vi "SaveMeasurement.vi"(8 "references":T1, 11 "measurement":T2) -> (0 "references out":T1, 3 "data":string[](array[string]))   [LabVIEW 2011]
doc: "Save measured data into the temporary .csv file for the case of program error."
uses:
  Measurement References.ctl
  <vilib>/Utility/NIReport.llb/NI_report.lvclass
  <vilib>/Utility/file.llb/Write To Spreadsheet File (string).vi
  <vilib>/Analysis/NI_AALBase.lvlib
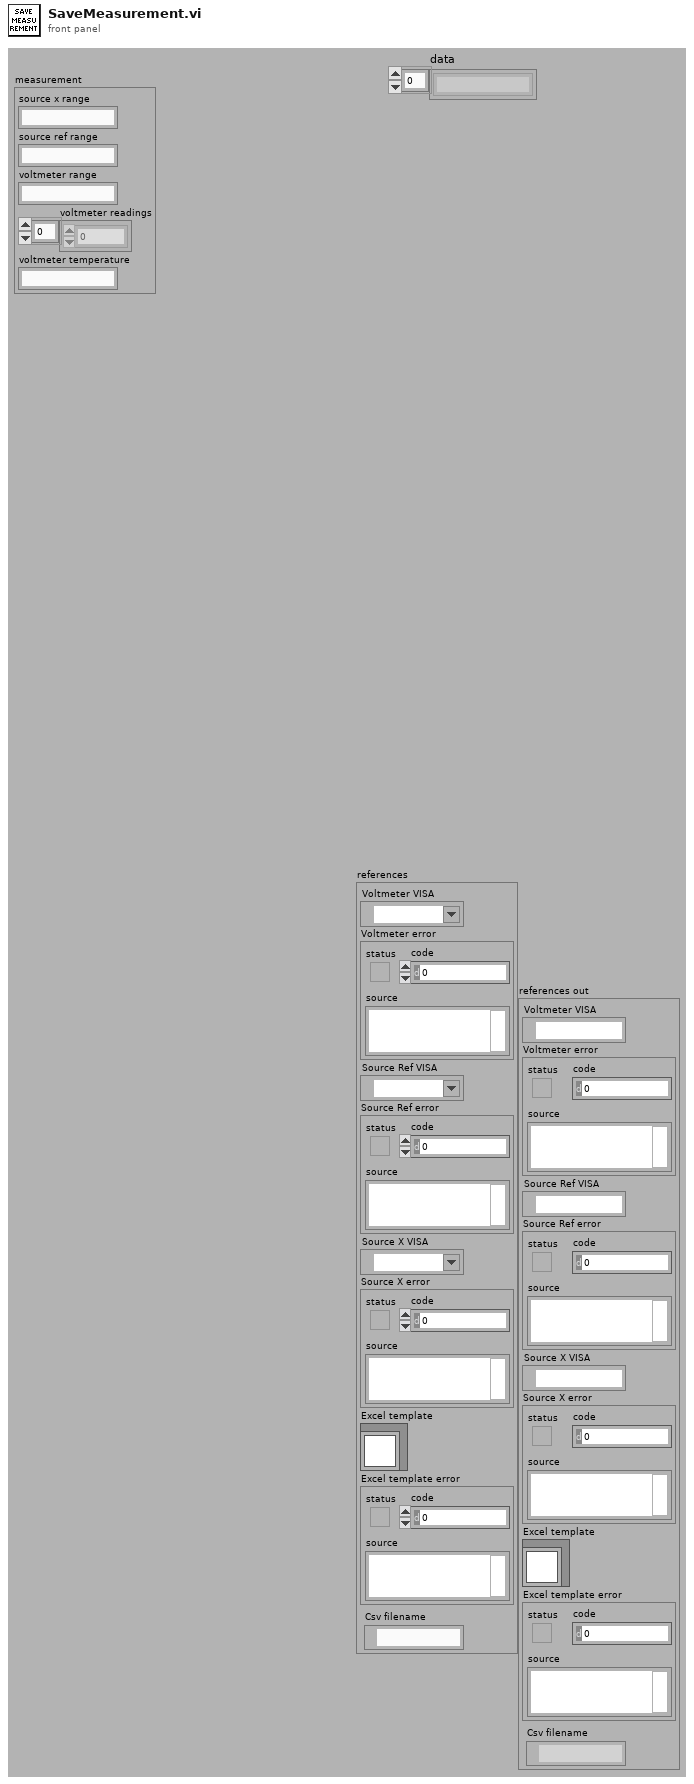
[diagram p1: front panel]
types:
  T1 = typedef "Measurement References.ctl" = cluster{"Voltmeter VISA":refnum<visa-resource-name>, "Voltmeter error":errorcluster, "Source Ref VISA":refnum<visa-resource-name>, "Source Ref error":errorcluster, "Source X VISA":refnum<visa-resource-name>, "Source X error":errorcluster, "Excel template":refnum<class "NI_report.lvclass">, "Excel template error":errorcluster, "Csv filename":path}
  T2 = cluster{"source x range":string, "source ref range":string, "voltmeter range":string, "voltmeter readings":dbl[], "voltmeter temperature":string}
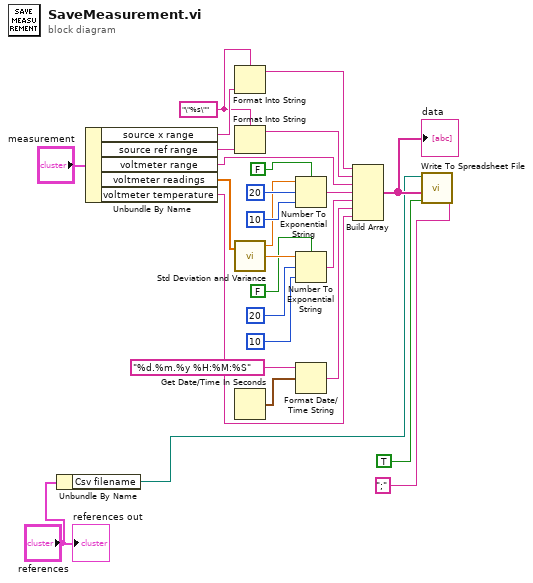
[diagram p0: block diagram]
diagram:
  w7 = "\"%s\"" ("format string")
  n1 = Unbundle By Name("references") -> ("Csv filename"=w1:path)
  n2 = Unbundle By Name("measurement") -> ("source x range"=w24:string, "source ref range"=w25:string, "voltmeter range"=w26:string, "voltmeter readings"=w9:dbl[], "voltmeter temperature"=w27:string)
  n3 = Format Into String(format string=w7, w24) -> (resulting string=w6:string)  [unwired: 2 in, 1 out]
  n4 = Format Into String(format string=w7, w25) -> (resulting string=w5:string)  [unwired: 2 in, 1 out]
  n5 = call <vilib>:"Std Deviation and Variance.vi"("X"=w9) -> ("mean"=w10:dbl, "standard deviation"=w17:dbl)  [unwired: 1 in, 1 out]
  n6 = Get Date/Time In Seconds() -> (seconds since 1Jan1904=w20:timestamp)
  n7 = Number To Exponential String(number=w10, precision (6)=i16 10, 1:FALSE ("use system decimal point (T)"), 3:i16 20 ("width (-)")) -> (E-format string=w18:string)
  n8 = Number To Exponential String(number=w17, precision (6)=i16 10, 1:FALSE ("use system decimal point (T)"), 3:i16 20 ("width (-)")) -> (E-format string=w19:string)
  n9 = Format Date/Time String(time format string (%c)="%d.%m.%y %H:%M:%S", seconds (now)=w20) -> (date/time string=w22:string)  [unwired: 1 in]
  n10 = Build Array(w6, w5, w26, w18, w19, w22, w27) -> (w8:string[])
  "data" <- w8
  n11 = call-poly <vilib>:"Write To Spreadsheet File.vi"("delimiter (\\t)"=";" ("delimiter (\\t)"), "append to file? (new file:F)"=TRUE, "1D data"=w8, "file path (dialog if empty)"=w1) -> ()  [unwired: 4 in, 1 out]
  "references out" <- "references"
